vi "AI Base Initialize.vi"(0 "OpenAI API URL":string caption="OpenAI API URL (e.g. OpenRouter, LM Studio)", 1 "Python venv path":path, 5 "API Key":string, 9 "Python version":string, 11 "error in (no error)":errorcluster, 12 "Anaconda path":path, 13 "conda env name":string) -> (4 "Python Refnum out":refnum<k35>, 10 "Http Client Handle out":T1, 15 "error out":errorcluster)   [LabVIEW 2023, in "LabVIEW AI Base.lvlib"]
uses:
  LabVIEW AI Base.lvlib
  <vilib>/httpClient/ClientHandle.ctl
  <vilib>/Utility/error.llb/Trim Whitespace One-Sided.vi
  AI Base Globals.vi
  <vilib>/Python/Open Venv Python Session.vi
  <vilib>/Python/Open Anaconda Python Session.vi
  <vilib>/httpClient/LabVIEWHTTPClient.lvlib
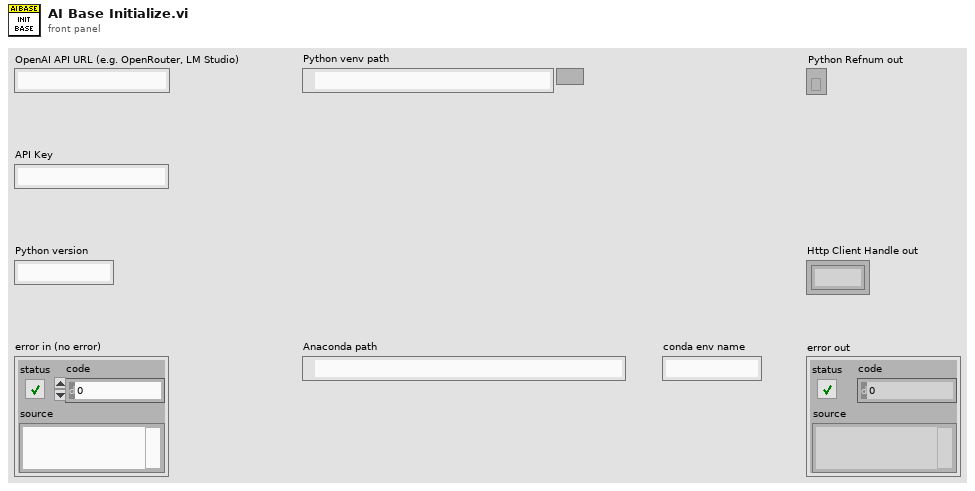
[diagram p1: front panel]
types:
  T1 = typedef "LabVIEWHTTPClient.lvlib/ClientHandle.ctl" = refnum<k1>
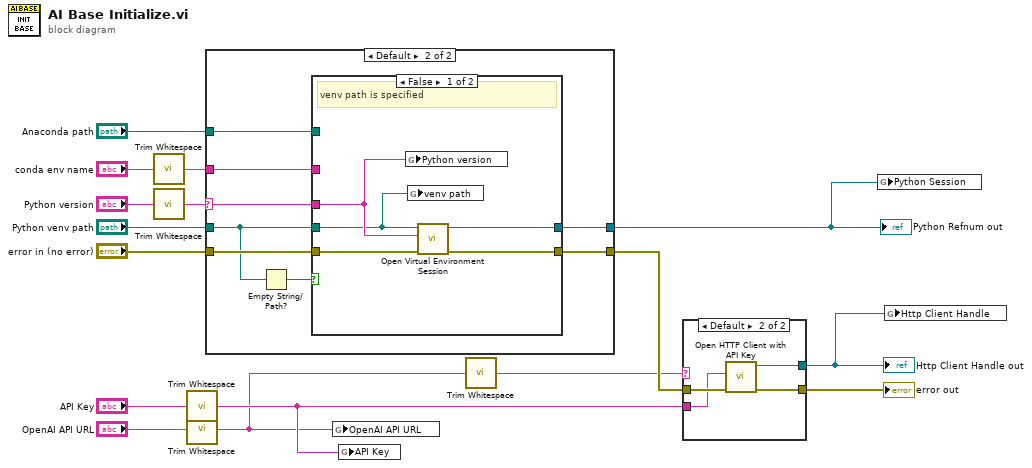
[diagram p0: block diagram]
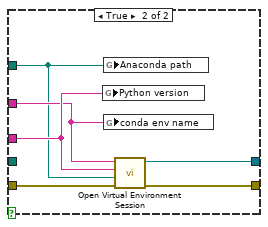
[diagram p4: hidden frame]
diagram:
  n1 = call <vilib>:"Trim Whitespace.vi"("string"="conda env name") -> ("trimmed string"=w1:string)  [unwired: 1 in]
  n2 = call <vilib>:"Trim Whitespace.vi"("string"="Python version") -> ("trimmed string"=w7:string)  [unwired: 1 in]
  n3 = call <vilib>:"Trim Whitespace.vi"("string"="API Key") -> ("trimmed string"=w3:string)  [unwired: 1 in]
  n4 = call <vilib>:"Trim Whitespace.vi"("string"="OpenAI API URL") -> ("trimmed string"=w2:string)  [unwired: 1 in]
  n5 = case shown="Default" w7 {
    selector: w7 -> [_ w24]
    tunnel: [w17 w25] -> w16
    tunnel: "error in (no error)" -> [w17 w23]
    tunnel: "Python venv path" -> [_ w21]
    tunnel: "Anaconda path" -> [_ w20]
    tunnel: w1 -> [_ w19]
    tunnel: [_ w18] -> w9
    frame "" {
    }
    frame Default {
      n6 = Empty String/Path?(string/path=w21) -> (empty?=w22:bool)
      n7 = case shown="False" w22 {
        tunnel: [w30 w36] -> w18
        tunnel: [w29 w35] -> w25
        tunnel: w24 -> [w28 w34]
        tunnel: w23 -> [w27 w33]
        tunnel: w21 -> [w26 _]
        tunnel: w20 -> [_ w31]
        tunnel: w19 -> [_ w32]
        frame False {
          # "venv path is specified"
          n8 = global write "AI Base Globals.vi" "Python version"(w28) -> ()
          n9 = global write "AI Base Globals.vi" "venv path"(w26) -> ()
          n10 = call-poly <vilib>:"Open Virtual Environment Session.vi"("error in (no error)"=w27, "Python version"=w28, "Env path"=w26) -> ("error out"=w29:errorcluster, "session out"=w30:refnum<k35>)  [unwired: 7 in]
        }
        frame True {
          n11 = global write "AI Base Globals.vi" "Python version"(w34) -> ()
          n12 = global write "AI Base Globals.vi" "Anaconda path"(w31) -> ()
          n13 = global write "AI Base Globals.vi" "conda env name"(w32) -> ()
          n14 = call-poly <vilib>:"Open Virtual Environment Session.vi"("error in (no error)"=w33, "Anaconda path"=w31, "Python version"=w34, "Env name"=w32) -> ("error out"=w35:errorcluster, "session out"=w36:refnum<k35>)  [unwired: 6 in]
        }
      }
    }
  }
  "Python Refnum out" <- w9
  n15 = global write "AI Base Globals.vi" "OpenAI API URL"(w2) -> ()
  n16 = global write "AI Base Globals.vi" "API Key"(w3) -> ()
  n17 = call <vilib>:"Trim Whitespace.vi"("string"=w2) -> ("trimmed string"=w6:string)  [unwired: 1 in]
  n18 = case shown="Default" w6 {
    tunnel: w16 -> [w37 w41]
    tunnel: [w37 w40] -> w15
    tunnel: [_ w39] -> w8
    tunnel: w3 -> [_ w38]
    frame "" {
    }
    frame Default {
      n19 = call "Open HTTP Client with API Key.vi"("error in"=w41, "API Key"=w38) -> ("error out"=w40:errorcluster, "Refnum out"=w39:T1)  [unwired: 8 in]
    }
  }
  "error out" <- w15
  "Http Client Handle out" <- w8
  n20 = global write "AI Base Globals.vi" "Python Session"(w9) -> ()
  n21 = global write "AI Base Globals.vi" "Http Client Handle"(w8) -> ()
